vi "SelectChildTag.vi"(7 "LoopData in":T2, 10 "Name":string, 11 "TagPath in":string[](array[string])) -> (2 "Item":T1, 3 "TagPath out":string[](array[string]), 5 "LoopData out":T2)   [LabVIEW 2020, in "BlueVariantView.lvlib"]
uses:
  BlueVariantView.lvlib
  LoopData.ctl
  API/Typedefs/TreeData.ctl
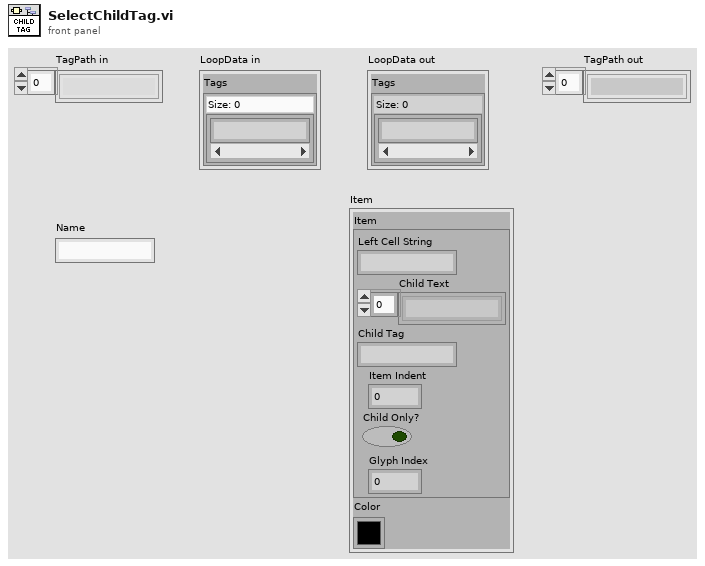
[diagram p1: front panel]
types:
  T1 = typedef "BlueVariantView.lvlib/TreeData.ctl" = cluster{"Item":cluster{"Left Cell String":string, "Child Text":string[], "Child Tag":string, "Item Indent":i32, "Child Only?":bool, "Glyph Index":i32}, "Color":u32}
  T2 = typedef "BlueVariantView.lvlib/LoopData.ctl" = cluster{"Tags":set{string}}
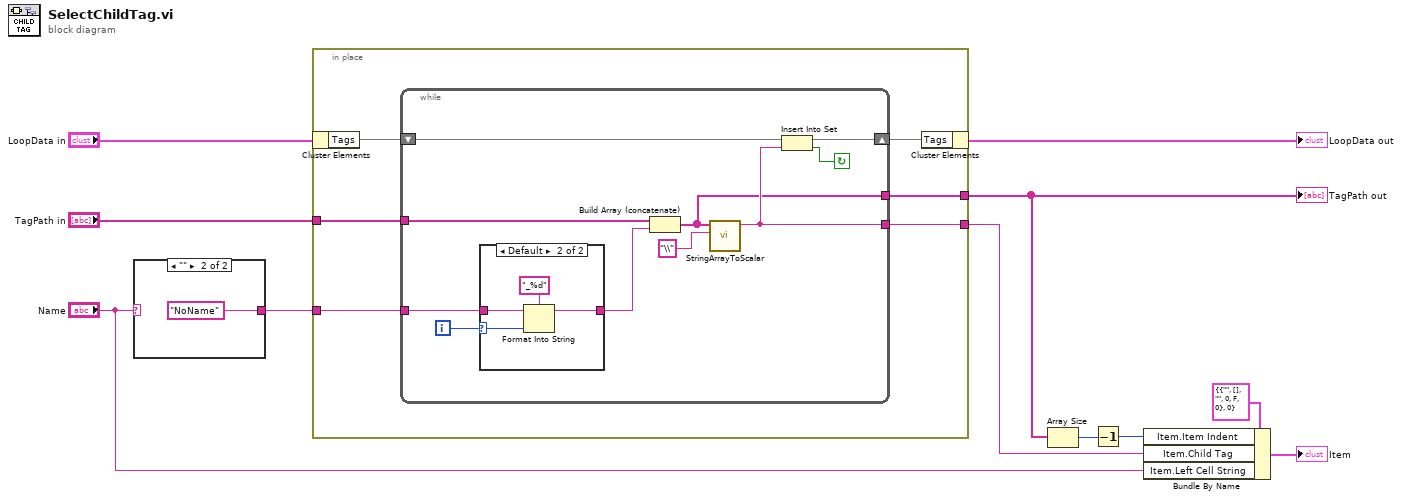
[diagram p0: block diagram]
diagram:
  n1 = case shown="\"\"" "Name" {
    selector: "Name" -> [w12 _]
    tunnel: [w12 "NoName"] -> w6
    frame Default {
    }
    frame "" {
    }
  }
  n2 = in-place {
    in-place-border: "TagPath in" -> [w19]
    in-place-border: w6 -> [w18]
    in-place-border: [w15] -> w5
    in-place-border: [w14] -> w8
    n3 = in-place-cluster #1("LoopData in") -> ("Tags"=w17:set{string})
    n4 = while {
      tunnel: w19 -> [w29]
      tunnel: w18 -> [w24]
      shift-right: [w27] -> w16
      shift-left: w17 -> [w28]
      tunnel: [w21] -> w15
      tunnel: [w20] -> w14
      i -> [w25]
      stop <- w26 continue-if-true
      n5 = case shown="Default" w25 {
        selector: w25 -> [_ w32]
        tunnel: w24 -> [w30 w33]
        tunnel: [w30 w31] -> w23
        frame 0 {
        }
        frame Default {
          n6 = Format Into String(format string="_%d", initial string=w33, w32) -> (resulting string=w31:string)  [unwired: 1 in, 1 out]
        }
      }
      n7 = Build Array (concatenate)(w29, w23) -> (w20:string[])
      n8 = call "StringArrayToScalar.vi"("delimiter (\\)"="\\" ("delimiter (\\)"), "Array"=w20) -> ("String"=w21:string)  [unwired: 9 in]
      n9 = Insert Into Set(10:w21, 11:w28) -> (2:w26:bool, 3:w27:set{string})
    }
    n10 = in-place-cluster #1("Tags"=w16) -> (→"LoopData out":T2)
  }
  "TagPath out" <- w8
  n11 = Array Size(array=w8) -> (size(s)=w4:i32)
  n12 = Decrement(x=w4) -> (x-1=w3:i32)
  n13 = Bundle By Name(cluster=T1 {"Item"={"Left Cell String"="", "Child Text"=[], "Child Tag"="", "Item Indent"=0, "Child Only?"=FALSE, "Glyph Index"=0}, "Color"=0} ("Cluster"), "Item.Item Indent"=w3, "Item.Child Tag"=w5, "Item.Left Cell String"="Name") -> (→"Item":T1)
